vi "Comptage 9425-4.vi"() -> ()   [LabVIEW 2022 SP3]
uses:
  <vilib>/Platform/TimedLoop/XDataNode/timing_clust.ctl
  <vilib>/Platform/TimedLoop/XDataNode/nitl_modes.ctl
  <vilib>/Platform/TimedLoop/XDataNode/wakeup.ctl
  <vilib>/DAQmx/read.llb/DAQmx Read (Digital 2D U32 NChan NSamp).vi
  Variables globales/Variable globale compteurs.vi
  Variables globales/Variable glob generale.vi
  <vilib>/DAQmx/miscellaneous.llb/DAQmx Fill In Error Info.vi
  <vilib>/Platform/TimedLoop/XDataNode/XDataNode.xnode
  <vilib>/Platform/TimedLoop/XDataNode/XDNodeRunTimeDep.lvlib
panel:
  out "Data compteurs":string[](array[string])
  # "NI-9425"
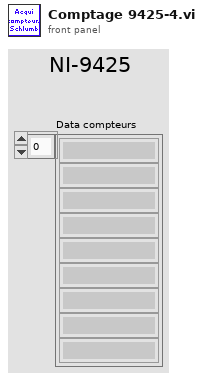
[diagram p1: front panel]
types:
  T1 = cluster{"Nom tache compteurs":refnum<k21>, "Noms des compteurs":string[], "Selection":bool[], "Init compteurs":dbl[], "Noms compteurs selectionnes":string[]}
  T2 = typedef "XDNodeRunTimeDep.lvlib/timing_clust.ctl" = cluster{"Expected End [f-1]":u64, "Actual End [f-1]":u64, "Finished Late? [f-1]":bool, "Expected End [i-1]":u64, "Actual End [i-1]":u64, "Finished Late? [i-1]":bool, "Expected Start [i]":u64, "Actual Start [i]":u64, "Expected Start [f]":u64, "Actual Start [f]":u64, "Source Name":string, "Structure Name":string, "Period":i64, "Deadline":i64, "Offset":i64, "Start":i64, "Priority":i32, "Timeout":i32, "Mode":T3, "Wakeup Reason":T4, "Error":errorcluster, "Source Type":string, "Secondary Source Type":string, "Global End Time":u64, "Global Start Time":u64, "Frame Duration":u64, "Iteration Duration":u64, "Assigned CPU":i32, "I/O Scan Engine Mode":u32}
  T3 = typedef "XDNodeRunTimeDep.lvlib/nitl_modes.ctl" = enum32{"No Change", "Process missed periods, maintain original phase", "Discard missed periods, maintain original phase", "Process missed periods, ignore original phase", "Discard missed periods, ignore original phase"}
  T4 = typedef "XDNodeRunTimeDep.lvlib/wakeup.ctl" = enum32{"Normal", "Aborted", "Asynchronous wakeup", "Timing source error", "Timed loop error", "Timeout"}
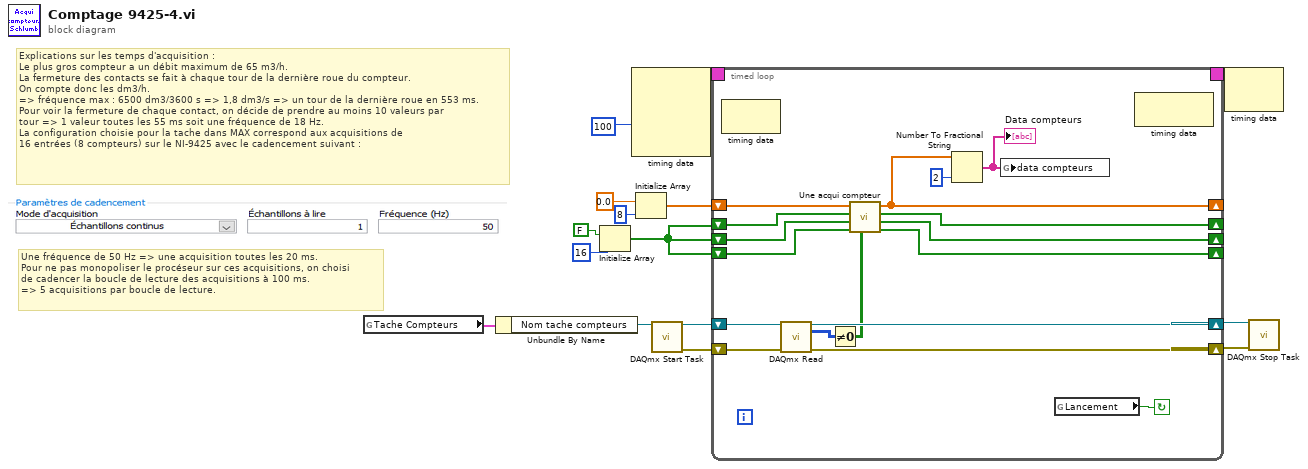
[diagram p0: block diagram]
diagram:
  # "Explications sur les temps d'acquisition :\nLe plus gros compteur a un débit maximum de 65 m3/h.\nLa fermeture des contacts se fait à chaque tour de la dernière roue du compteur.\nOn compte donc les dm3/h.\n=> fréquence max : 6500 dm3/3600 s => 1,8 dm3/s => un tour de la dernière roue en 553 ms.\nPour voir la fermeture de chaque contact, on décide de prendre au moins 10 valeurs par\ntour => 1 valeur toutes les 55 ms soit une fréquence de 18 Hz.\nLa configuration choisie pour la tache dans MAX correspond aux acquisitions de\n16 entrées (8 compteurs) sur le NI-9425 avec le cadencement suivant :"
  # "Une fréquence de 50 Hz => une acquisition toutes les 20 ms.\nPour ne pas monopoliser le procéseur sur ces acquisitions, on choisi \nde cadencer la boucle de lecture des acquisitions à 100 ms.\n=> 5 acquisitions par boucle de lecture."
  n1 = global read "Variable globale compteurs.vi" "Tache Compteurs"() -> (w2:T1)
  n2 = Unbundle By Name(w2) -> ("Nom tache compteurs"=w1:refnum<k21>)
  n3 = Initialize Array(FALSE, 16 ("taille de la dimension")) -> (w6:bool[])
  n4 = node-c288(i64 100 ("Période")) -> (w9:T2)  [unwired: 3 in]
  n5 = Initialize Array(0.0 ("élément"), 8 ("taille de la dimension")) -> (w4:dbl[])
  n6 = call <vilib>:"DAQmx Start Task.vi"("task/channels in"=w1) -> ("task out"=w15:refnum<k21>, "error out"=w14:errorcluster)  [unwired: 13 in]
  n7 = timed-loop {
    shift-right: [w30] -> w13
    shift-left: w15 -> [w32]
    shift-right: [w29] -> w12
    shift-left: w14 -> [w31]
    shift-right: [w18] -> _
    shift-left: w4 -> [w28]
    shift-right: [w23] -> _
    shift-left: w6 -> [w26]
    timing: w9 -> [_]
    timing-out: [_] -> w8
    shift-right: [w22] -> _
    shift-left: w6 -> [w25]
    shift-right: [w24] -> _
    shift-left: w6 -> [w27]
    stop <- w19 continue-if-true
    n8 = node-c288() -> ()  [unwired: 1 in, 1 out]
    n9 = call-poly <vilib>:"DAQmx Read.vi"("task/channels in"=w32, "error in"=w31) -> ("task out"=w30:refnum<k21>, "data"=w20:u32[][], "error out"=w29:errorcluster)  [unwired: 11 in]
    n10 = Not Equal To 0?(x=w20) -> (x != 0?=w21:bool[][])
    n11 = call "Une acqui compteur.vi"("entrées"=w21, "BF2 i-1"=w25, "BF1 i-1"=w26, "s-1"=w27, "Valeurs compteur i-1"=w28) -> ("BF2 i"=w22:bool[], "BF1 i"=w23:bool[], "S"=w24:bool[], "Valeur compteur"=w18:dbl[])
    n12 = Number To Fractional String(number=w18, precision (6)=i16 2 ("précision (6)")) -> (F-format string=w16:string[])  [unwired: 2 in]
    "Data compteurs" <- w16
    n13 = global write "Variable globale compteurs.vi" "data compteurs"(w16) -> ()
    n14 = global read "Variable glob generale.vi" "Lancement"() -> (w19:bool)
    n15 = node-c288() -> ()  [unwired: 1 in, 1 out]
  }
  n16 = node-c288(w8) -> ()  [unwired: 1 out]
  n17 = call <vilib>:"DAQmx Stop Task.vi"("task/channels in"=w13, "error in"=w12) -> ()  [unwired: 12 in, 2 out]
